vi "W32B Parse Spec.vi"(0 "function name":string, 5 "library path":path, 7 "parameters":string, 9 "links":string, 11 "error in":errorcluster) -> (4 "CLFN":T2, 6 "links out":T1(array[cluster]), 15 "error out":errorcluster)   [LabVIEW 2020]
doc: "Turns the text spec of one wrapper into the CLFN cluster and links array W32B Build Wrapper.vi takes. parameters: one line per CLFN parameter - the FIRST line is the return value - as name;Parameter Type;Numeric Type;Param Passing;Adapt Format[;Num Dimensions] with enum INDICES (Parameter Type 0 Numeric, 1 Array, 7 Any/adapt to type. Numeric Type 2 I32, 5 U16, 6 U32, 10 PTR INT, 11 PTR UINT. Param Passing 0 by value, 1 pointer to value. Adapt Format 0 handles by value. Num Dimensions is optional and only needed for an array parameter - 1 for a 1D array. A seventh field Array Passing is optional too: 0 Array Data Pointer (default), 1 Array Handle, 2 Array Handle Pointer). links: one line per wire as CLFN terminal;control label;node class;node source (1 output, 0 input)."
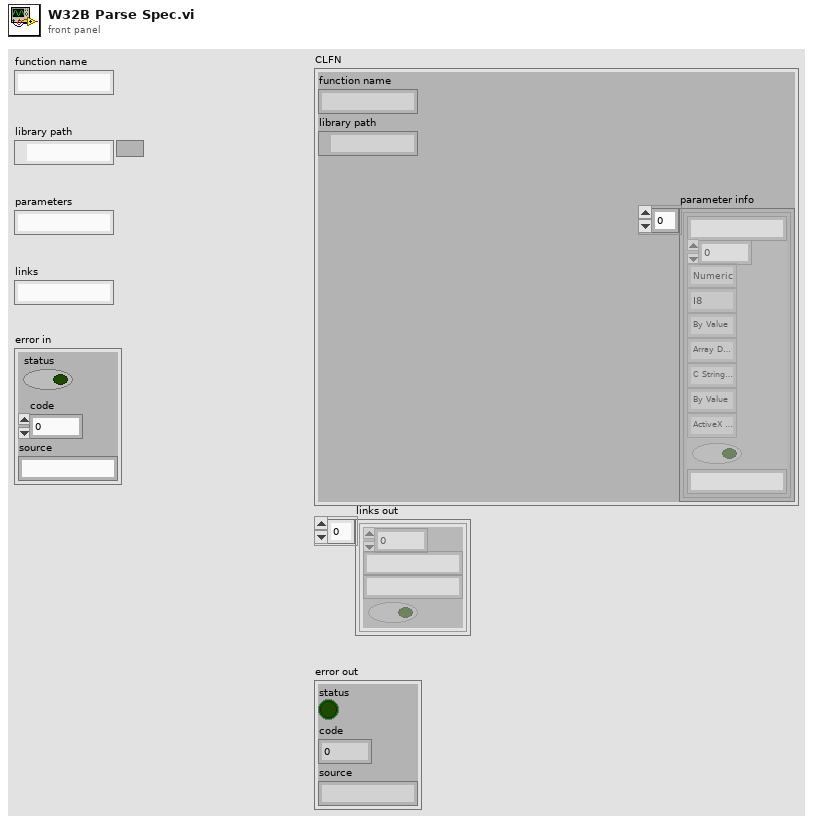
[diagram p1: front panel]
types:
  T1 = cluster{"CLFN terminal":i32, "control label":string, "node class":string, "node source?":bool}[]
  T2 = cluster{"function name":string, "library path":path, "parameter info":cluster{"Parameter Name":string, "Num Dimensions":i32, "Parameter Type":enum16{"Numeric", "Array", "String", "Waveform", "Digital Waveform", "Digital Table", "ActiveX", "Any", "Instance Data Pointer", "Void"}, "Numeric Type":enum16{"I8", "I16", "I32", "I64", "U8", "U16", "U32", "U64", "SGL", "DBL", "PTR INT", "PTR UINT"}, "Param Passing":enum16{"By Value", "Pointer To Value"}, "Array Passing":enum16{"Array Data Pointer", "Array Handle", "Array Handle Pointer"}, "String Passing":enum16{"C String Pointer", "Pascal String Pointer", "String Handle", "String Handle Pointer"}, "Adapt Format":enum16{"By Value", "Pointer To Value"}, "ActiveX Types":enum16{"ActiveX Variant Pointer", "IDispatch* Pointer", "IUnknown* Pointer"}, "Const (unused)":bool, "Minimum Size":string}[]}
  T3 = cluster{"CLFN terminal":i32, "control label":string, "node class":string, "node source?":bool}
  T4 = cluster{"Parameter Name":string, "Num Dimensions":i32, "Parameter Type":enum16{"Numeric", "Array", "String", "Waveform", "Digital Waveform", "Digital Table", "ActiveX", "Any", "Instance Data Pointer", "Void"}, "Numeric Type":enum16{"I8", "I16", "I32", "I64", "U8", "U16", "U32", "U64", "SGL", "DBL", "PTR INT", "PTR UINT"}, "Param Passing":enum16{"By Value", "Pointer To Value"}, "Array Passing":enum16{"Array Data Pointer", "Array Handle", "Array Handle Pointer"}, "String Passing":enum16{"C String Pointer", "Pascal String Pointer", "String Handle", "String Handle Pointer"}, "Adapt Format":enum16{"By Value", "Pointer To Value"}, "ActiveX Types":enum16{"ActiveX Variant Pointer", "IDispatch* Pointer", "IUnknown* Pointer"}, "Const (unused)":bool, "Minimum Size":string}
  T5 = cluster{"function name":string, "library path":path, cluster{"Parameter Name":string, "Num Dimensions":i32, "Parameter Type":enum16{"Numeric", "Array", "String", "Waveform", "Digital Waveform", "Digital Table", "ActiveX", "Any", "Instance Data Pointer", "Void"}, "Numeric Type":enum16{"I8", "I16", "I32", "I64", "U8", "U16", "U32", "U64", "SGL", "DBL", "PTR INT", "PTR UINT"}, "Param Passing":enum16{"By Value", "Pointer To Value"}, "Array Passing":enum16{"Array Data Pointer", "Array Handle", "Array Handle Pointer"}, "String Passing":enum16{"C String Pointer", "Pascal String Pointer", "String Handle", "String Handle Pointer"}, "Adapt Format":enum16{"By Value", "Pointer To Value"}, "ActiveX Types":enum16{"ActiveX Variant Pointer", "IDispatch* Pointer", "IUnknown* Pointer"}, "Const (unused)":bool, "Minimum Size":string}[]}
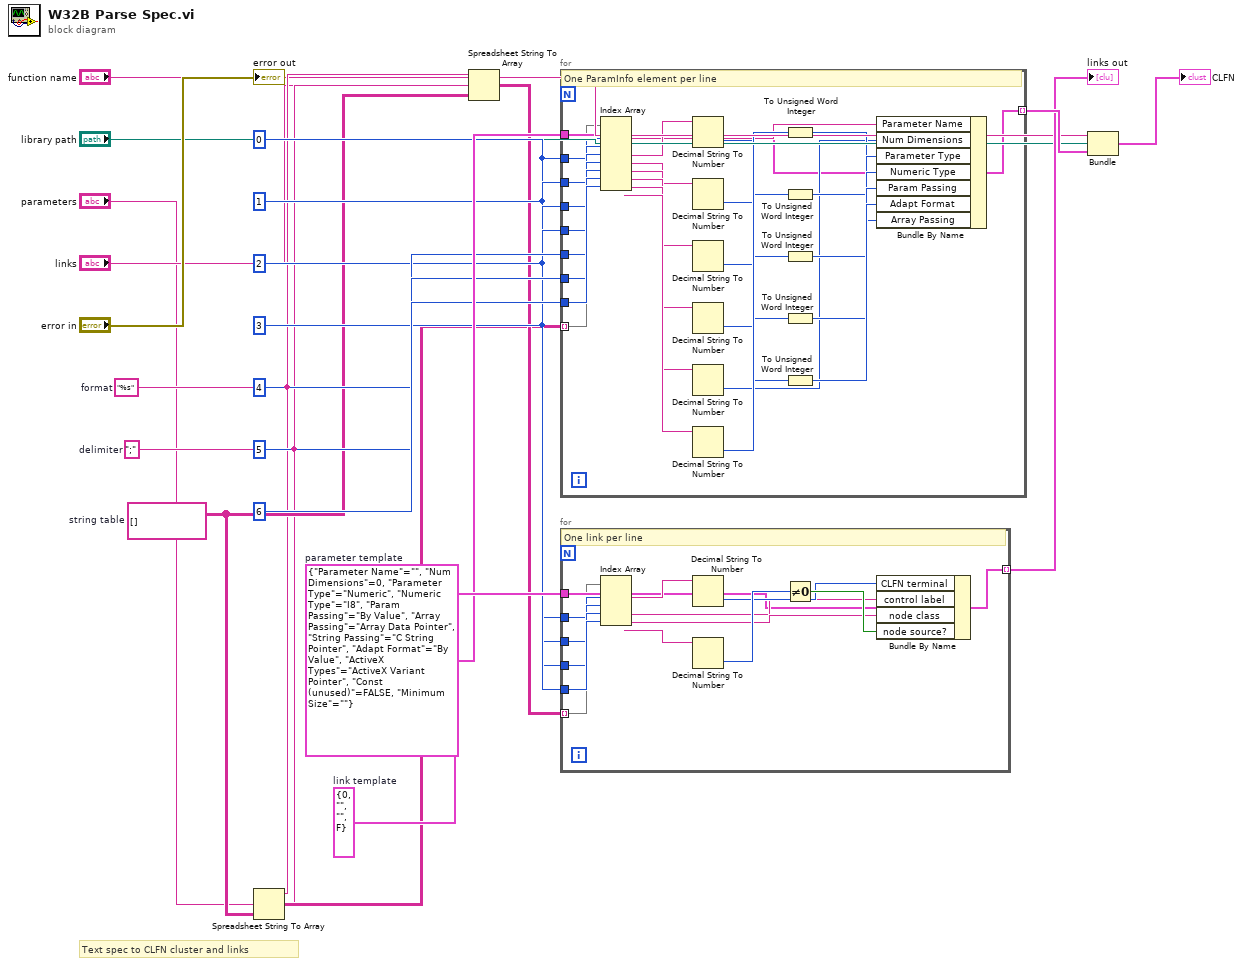
[diagram p0: block diagram]
diagram:
  w21 = T3 {"CLFN terminal"=0, "control label"="", "node class"="", "node source?"=FALSE}  # link template
  w20 = T4 {"Parameter Name"="", "Num Dimensions"=0, "Parameter Type"=enum."Numeric", "Numeric Type"=enum."I8", "Param Passing"=enum."By Value", "Array Passing"=enum."Array Data Pointer", "String Passing"=enum."C String Pointer", "Adapt Format"=enum."By Value", "ActiveX Types"=enum."ActiveX Variant Pointer", "Const (unused)"=FALSE, "Minimum Size"=""}  # parameter template
  w16 = 3
  w15 = 2
  w14 = 1
  w13 = 0
  w10 = string[][] []  # string table
  w9 = ";"  # delimiter
  w8 = "%s"  # format
  # "Text spec to CLFN cluster and links"
  n1 = Spreadsheet String To Array(delimiter (Tab)=w9, format string=w8, spreadsheet string="parameters", array type (2D Dbl)=w10) -> (array=w11:string[][])
  n2 = Spreadsheet String To Array(delimiter (Tab)=w9, format string=w8, spreadsheet string="links", array type (2D Dbl)=w10) -> (array=w12:string[][])
  n3 = for {
    tunnel: w20 -> [w24]
    tunnel: w13 -> [w25]
    tunnel: w14 -> [w26]
    tunnel: w15 -> [w27]
    tunnel: w16 -> [w28]
    tunnel: 4 -> [w29]
    tunnel: 5 -> [w30]
    tunnel: 6 -> [w31]
    tunnel: w11 -> [w23] mode=indexing
    tunnel: [w50] -> w22 mode=indexing
    # "One ParamInfo element per line"
    n4 = Index Array(array=w23, index #1=w25, index #2=w26, index #3=w27, index #4=w28, index #5=w29, index #6=w30, index #7=w31) -> (element #1=w32:string, element #2=w33:string, element #3=w34:string, element #4=w35:string, element #5=w36:string, element #6=w37:string, element #7=w38:string)
    n5 = Decimal String To Number(string=w33) -> (number=w39:i32)  [unwired: 2 in, 1 out]
    n6 = Decimal String To Number(string=w34) -> (number=w40:i32)  [unwired: 2 in, 1 out]
    n7 = Decimal String To Number(string=w35) -> (number=w41:i32)  [unwired: 2 in, 1 out]
    n8 = Decimal String To Number(string=w36) -> (number=w42:i32)  [unwired: 2 in, 1 out]
    n9 = Decimal String To Number(string=w37) -> (number=w43:i32)  [unwired: 2 in, 1 out]
    n10 = Decimal String To Number(string=w38) -> (number=w44:i32)  [unwired: 2 in, 1 out]
    n11 = To Unsigned Word Integer(number=w44) -> (unsigned 16bit integer=w45:u16)
    n12 = To Unsigned Word Integer(number=w39) -> (unsigned 16bit integer=w46:u16)
    n13 = To Unsigned Word Integer(number=w40) -> (unsigned 16bit integer=w47:u16)
    n14 = To Unsigned Word Integer(number=w41) -> (unsigned 16bit integer=w48:u16)
    n15 = To Unsigned Word Integer(number=w42) -> (unsigned 16bit integer=w49:u16)
    n16 = Bundle By Name(cluster=w24, "Parameter Name"=w32, "Num Dimensions"=w43, "Parameter Type"=w46, "Numeric Type"=w47, "Param Passing"=w48, "Adapt Format"=w49, "Array Passing"=w45) -> (w50:T4)
  }
  n17 = for {
    tunnel: w21 -> [w52]
    tunnel: w13 -> [w53]
    tunnel: w14 -> [w54]
    tunnel: w15 -> [w55]
    tunnel: w16 -> [w56]
    tunnel: w12 -> [w51] mode=indexing
    tunnel: [w64] -> w7 mode=indexing
    # "One link per line"
    n18 = Index Array(array=w51, index #1=w53, index #2=w54, index #3=w55, index #4=w56) -> (element #1=w57:string, element #2=w58:string, element #3=w59:string, element #4=w60:string)
    n19 = Decimal String To Number(string=w57) -> (number=w61:i32)  [unwired: 2 in, 1 out]
    n20 = Decimal String To Number(string=w60) -> (number=w62:i32)  [unwired: 2 in, 1 out]
    n21 = Not Equal To 0?(x=w62) -> (x != 0?=w63:bool)
    n22 = Bundle By Name(cluster=w52, "CLFN terminal"=w61, "control label"=w58, "node class"=w59, "node source?"=w63) -> (w64:T3)
  }
  "links out" <- w7
  n23 = Bundle("function name"="function name", "library path"="library path", w22) -> (→"CLFN":T5)  [unwired: 1 in]
  "error out" <- "error in"
